vi "Revert to Scan Mode.vi"(8 "error in":errorcluster) -> (0 "error out":errorcluster)   [LabVIEW 2027, in "SEECD System Explorer.lvlib"]
uses:
  SEECD System Explorer.lvlib
  C:/Program Files/dotnet/shared/Microsoft.NETCore.App/10.0.12/System.Private.CoreLib.dll
  Program Files/dotnet/shared/Microsoft.NETCore.App/10.0.12/System.Private.CoreLib.dll
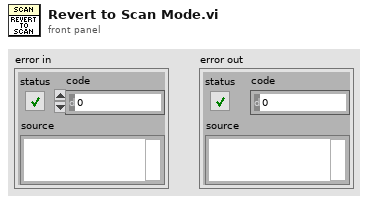
[diagram p1: front panel]
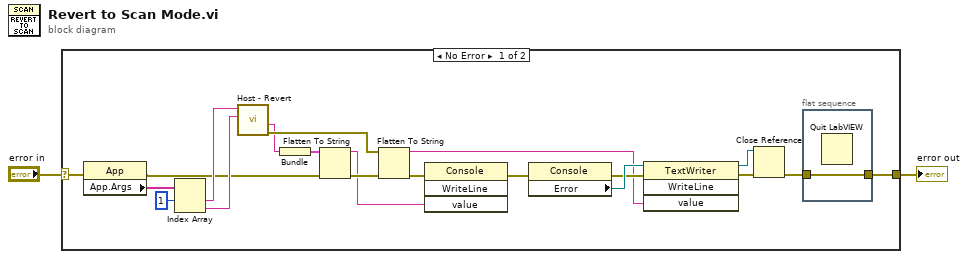
[diagram p0: block diagram]
diagram:
  n1 = case shown="No Error" "error in" {
    selector: "error in" -> [w22 w24]
    tunnel: [w20 w24] -> w1
    frame No Error {
      n2 = property class="App"(error in=w22) -> (error out=w6:errorcluster, "App.Args"=w10:string[])  [unwired: 1 in, 1 out]
      n3 = Index Array(array=w10, index #1=1 ("index")) -> (element #1=w12:string, element #2=w11:string)  [unwired: 1 in]
      n4 = call "Host - Revert.vi"("Target IP Address in"=w11, "Slave Ref in"=w12) -> ("error out"=w13:errorcluster, "Message output"=w5:string)  [unwired: 6 in, 2 out]
      n5 = Bundle("Message output"=w5) -> (w4:cluster{"Message output":string})  [unwired: 1 in]
      n6 = Flatten To String(anything=w4, error in (no error)=w6) -> (data string=w3:string, error out=w7:errorcluster)  [unwired: 2 in, 1 out]
      n7 = Flatten To String(anything=w13, error in (no error)=w7) -> (data string=w17:string, error out=w8:errorcluster)  [unwired: 2 in, 1 out]
      n8 = invoke class="Console" method="WriteLine"(error in=w8, "value"=w3) -> (error out=w9:errorcluster)  [unwired: 2 in, 3 out]
      n9 = property class="Console"(error in=w9) -> (error out=w18:errorcluster, "Error"=w19:refnum<k39>)  [unwired: 1 in, 1 out]
      n10 = invoke class="TextWriter" method="WriteLine"(reference=w19, error in=w18, "value"=w17) -> (reference out=w16:refnum<k39>, error out=w14:errorcluster)  [unwired: 1 in, 2 out]
      n11 = Close Reference(reference=w16, error in (no error)=w14) -> (error out=w15:errorcluster)
      n12 = flat-sequence {
        tunnel: w15 -> [w23]
        tunnel: [w23] -> w20
        frame #0 {
          n13 = Quit LabVIEW() -> ()  [unwired: 1 in]
        }
      }
    }
    frame Error {
    }
  }
  "error out" <- w1
